vi "Windfreak_frequency_shift.vi"() -> ()   [LabVIEW 2024]
panel:
  in  "VISA resource name":refnum<visa-resource-name>
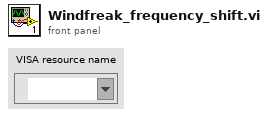
[diagram p1: front panel]
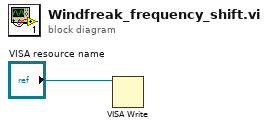
[diagram p0: block diagram]
diagram:
  n1 = VISA Write(VISA resource name="VISA resource name") -> ()  [unwired: 2 in, 3 out]
